vi "zad3.vi"() -> ()   [LabVIEW 2025]
uses:
  <vilib>/platform/TimedLoop/XDataNode/XDataNode.xnode
  <vilib>/Platform/TimedLoop/XDataNode/nitl_modes.ctl
  <vilib>/Platform/TimedLoop/XDataNode/XDNodeRunTimeDep.lvlib
  <vilib>/Platform/TimedLoop/XDataNode/wakeup.ctl
  <vilib>/Platform/TimedLoop/XDataNode/timing_clust.ctl
panel:
  in  "milliseconds to wait":u32
  in  "N":i32
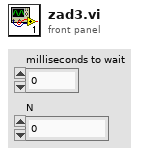
[diagram p1: front panel]
types:
  T1 = typedef "XDNodeRunTimeDep.lvlib/timing_clust.ctl" = cluster{"Expected End [f-1]":u64, "Actual End [f-1]":u64, "Finished Late? [f-1]":bool, "Expected End [i-1]":u64, "Actual End [i-1]":u64, "Finished Late? [i-1]":bool, "Expected Start [i]":u64, "Actual Start [i]":u64, "Expected Start [f]":u64, "Actual Start [f]":u64, "Source Name":string, "Structure Name":string, "Period":i64, "Deadline":i64, "Offset":i64, "Start":i64, "Priority":i32, "Timeout":i32, "Mode":T2, "Wakeup Reason":T3, "Error":errorcluster, "Source Type":string, "Secondary Source Type":string, "Global End Time":u64, "Global Start Time":u64, "Frame Duration":u64, "Iteration Duration":u64, "Assigned CPU":i32, "I/O Scan Engine Mode":u32}
  T2 = typedef "XDNodeRunTimeDep.lvlib/nitl_modes.ctl" = enum32{"No Change", "Process missed periods, maintain original phase", "Discard missed periods, maintain original phase", "Process missed periods, ignore original phase", "Discard missed periods, ignore original phase"}
  T3 = typedef "XDNodeRunTimeDep.lvlib/wakeup.ctl" = enum32{"Normal", "Aborted", "Asynchronous wakeup", "Timing source error", "Timed loop error", "Timeout"}
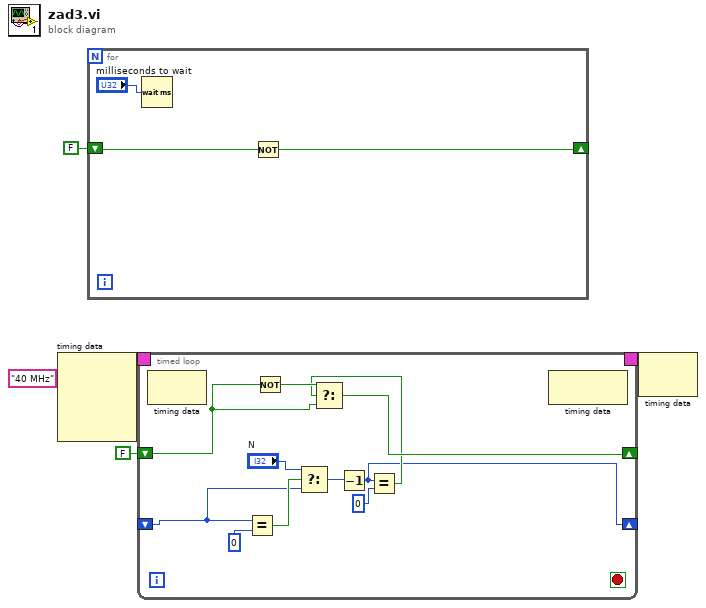
[diagram p0: block diagram]
diagram:
  n1 = node-c288("40 MHz" ("Source Name")) -> (w5:T1)  [unwired: 3 in]
  n2 = for {
    shift-right: [w7] -> _
    shift-left: FALSE -> [w6]
    n3 = Wait (ms)(milliseconds to wait="milliseconds to wait") -> ()  [unwired: 1 out]
    n4 = Not(x=w6) -> (.not. x?=w7:bool)
  }
  n5 = timed-loop {
    timing: w5 -> [_]
    timing-out: [_] -> w4
    shift-right: [w18] -> _
    shift-left: FALSE -> [w17]
    shift-right: [w12] -> _
    shift-left: _ -> [w9]
    stop <- _ stop-if-true
    n6 = node-c288() -> ()  [unwired: 1 in, 1 out]
    n7 = Equal?(x=w9, y=0) -> (x = y?=w10:bool)
    n8 = Not(x=w17) -> (.not. x?=w19:bool)
    n9 = Select(t="N", s=w10, f=w9) -> (s? t:f=w15:i32)
    n10 = Decrement(x=w15) -> (x-1=w12:i32)
    n11 = Equal?(x=w12, y=0) -> (x = y?=w13:bool)
    n12 = Select(t=w19, s=w13, f=w17) -> (s? t:f=w18:bool)
    n13 = node-c288() -> ()  [unwired: 1 in, 1 out]
  }
  n14 = node-c288(w4) -> ()  [unwired: 1 out]
